vi "Machine DB info IV.vi"(11 "Ex ID":string) -> (1 "MachineDB GPSET":string[][](array[string]), 2 "found!":bool, 3 "Chip ID":string)   [LabVIEW 2018]
panel:
  out "Chip ID array":string[](array[string])
  out "Ex ID array":string[](array[string])
  out "数値":i32
  out "エラー出力":errorcluster
  in  "エラー入力":errorcluster
  out "取り除かれたパス":path
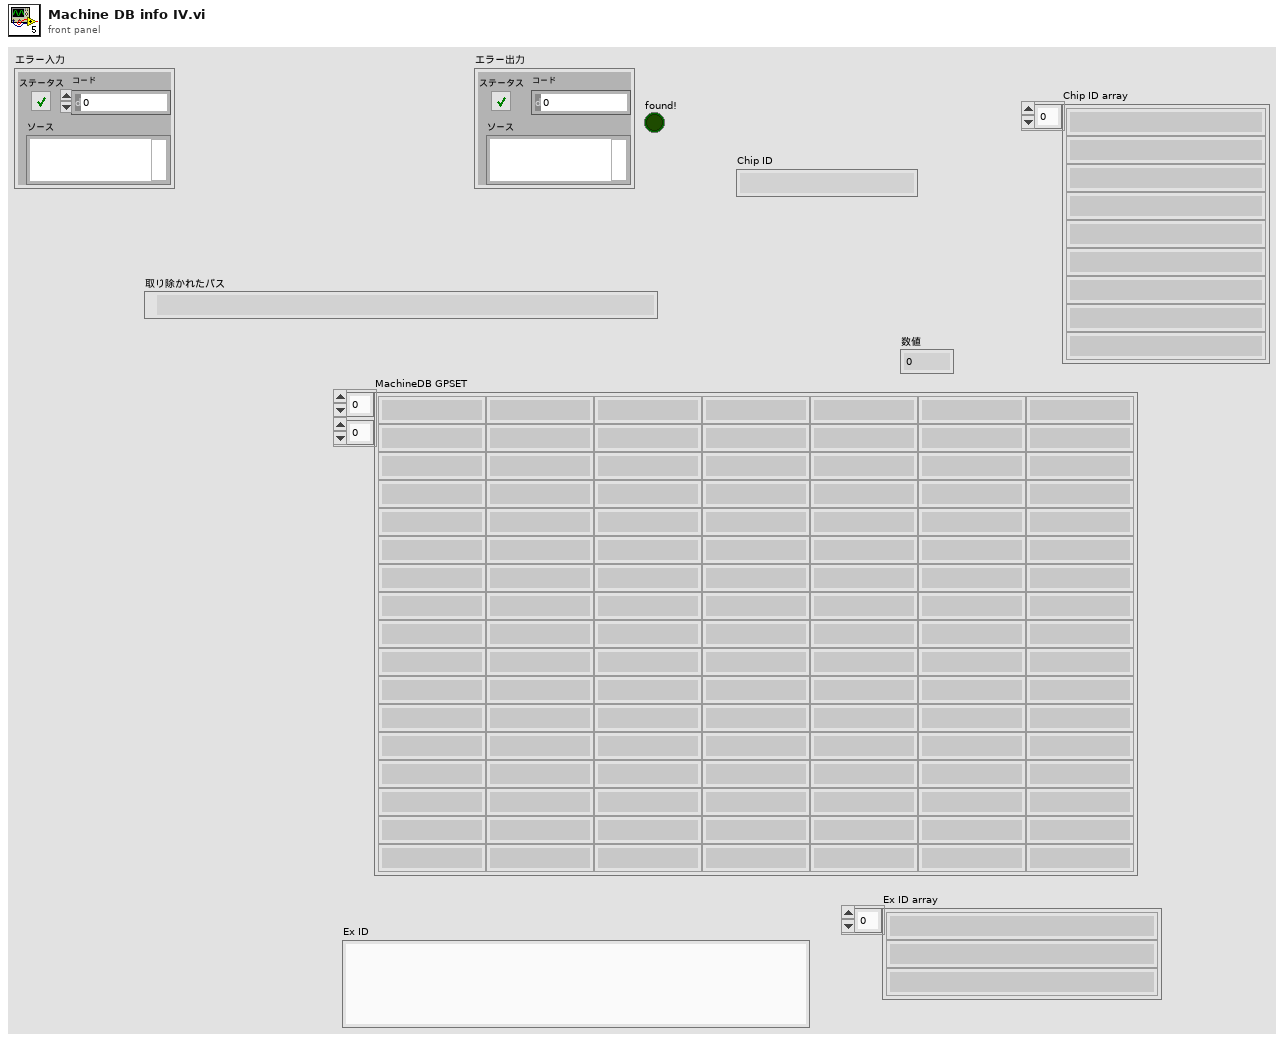
[diagram p1: front panel]
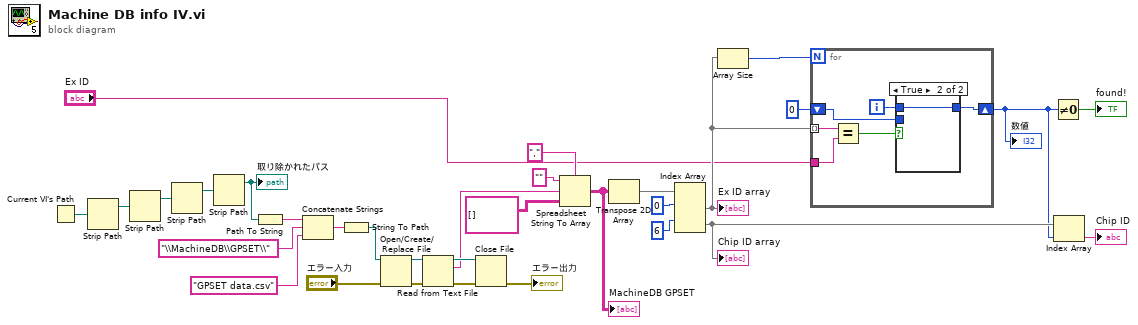
[diagram p0: block diagram]
diagram:
  n1 = Current VI's Path() -> (path=w32:path)
  n2 = Strip Path(path=w32) -> (stripped path=w31:path)  [unwired: 1 out]
  n3 = Strip Path(path=w31) -> (stripped path=w18:path)  [unwired: 1 out]
  n4 = Strip Path(path=w18) -> (stripped path=w17:path)  [unwired: 1 out]
  n5 = Strip Path(path=w17) -> (stripped path=w19:path)  [unwired: 1 out]
  "取り除かれたパス" <- w19
  n6 = Path To String(path=w19) -> (string=w30:string)
  n7 = Concatenate Strings(w30, "\\MachineDB\\GPSET\\" ("文字列"), "GPSET data.csv" ("文字列")) -> (w27:string)
  n8 = String To Path(string=w27) -> (path=w26:path)
  n9 = Open/Create/Replace File(file path (use dialog)=w26, error in="エラー入力") -> (refnum out=w24:refnum<file>, error out=w23:errorcluster)  [unwired: 4 in, 1 out]
  n10 = Read from Text File(file (use dialog)=w24, error in=w23) -> (refnum out=w22:refnum<file>, text=w15:string, error out=w21:errorcluster)  [unwired: 2 in, 1 out]
  n11 = Close File(refnum=w22, error in=w21) -> (error out=→"エラー出力":errorcluster)  [unwired: 1 out]
  n12 = Spreadsheet String To Array(delimiter (Tab)="," ("デリミタ（タブ）"), format string="" ("形式文字列"), spreadsheet string=w15, array type (2D Dbl)=string[][] []) -> (array=w11:string[][])
  "MachineDB GPSET" <- w11
  n13 = Transpose 2D Array(2D array=w11) -> (transposed array=w10:string[][])
  n14 = Index Array(array=w10, index (row) #1=0 ("指標 （行）"), index (row) #2=6 ("指標 （行）")) -> (element #1=w7:string[], element #2=w4:string[])  [unwired: 2 in]
  "Ex ID array" <- w7
  "Chip ID array" <- w4
  n15 = Array Size(array=w7) -> (size(s)=w9:i32)
  n16 = for {
    N: w9 -> [_]
    tunnel: w7 -> [w38] mode=indexing
    shift-right: [w36] -> w2
    shift-left: 0 -> [w35]
    tunnel: "Ex ID" -> [w34]
    i -> [w33]
    n17 = Equal?(x=w38, y=w34) -> (x = y?=w37:bool)
    n18 = case shown="True" w37 {
      tunnel: [w39 w40] -> w36
      tunnel: w35 -> [w39 _]
      tunnel: w33 -> [_ w40]
      frame False {
      }
      frame True {
      }
    }
  }
  "数値" <- w2
  n19 = Not Equal To 0?(x=w2) -> (x != 0?=→"found!":bool)
  n20 = Index Array(array=w4, index=w2) -> (element=→"Chip ID":string)
